vi "Test Assert Event to JSON.vi"(9 "indent level":i32, 10 "Test Event":T1={"Name"="", "Passed"=FALSE, "Call Chain"=[], "Test Error"={"status"=FALSE, "code"=0, "source"=""}, "Time Stamp"=timestamp(0 s since 1904-01-01), "Unique Assert ID"="", "Test ID"="", "Execution time (s)"=-1.0, "Verbose Explanation"=""}) -> (2 "<JSON>Assertion Event":string)   [LabVIEW 2020, in "Caraya.lvlib" / "Test Result.lvclass"]
uses:
  Test Result.lvclass
  Assert Event Data.ctl
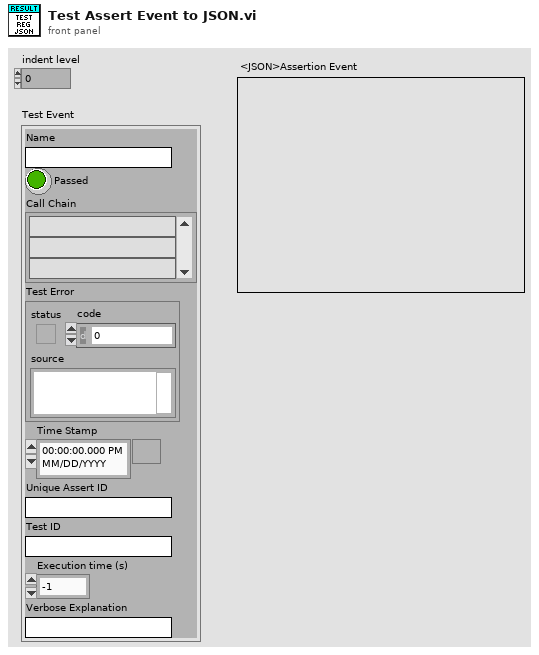
[diagram p1: front panel]
types:
  T1 = typedef "Caraya.lvlib/Test Result.lvclass/Assert Event Data.ctl" = cluster{"Name":string, "Passed":bool, "Call Chain":string[], "Test Error":errorcluster, "Time Stamp":timestamp, "Unique Assert ID":string, "Test ID":string, "Execution time (s)":dbl, "Verbose Explanation":string}
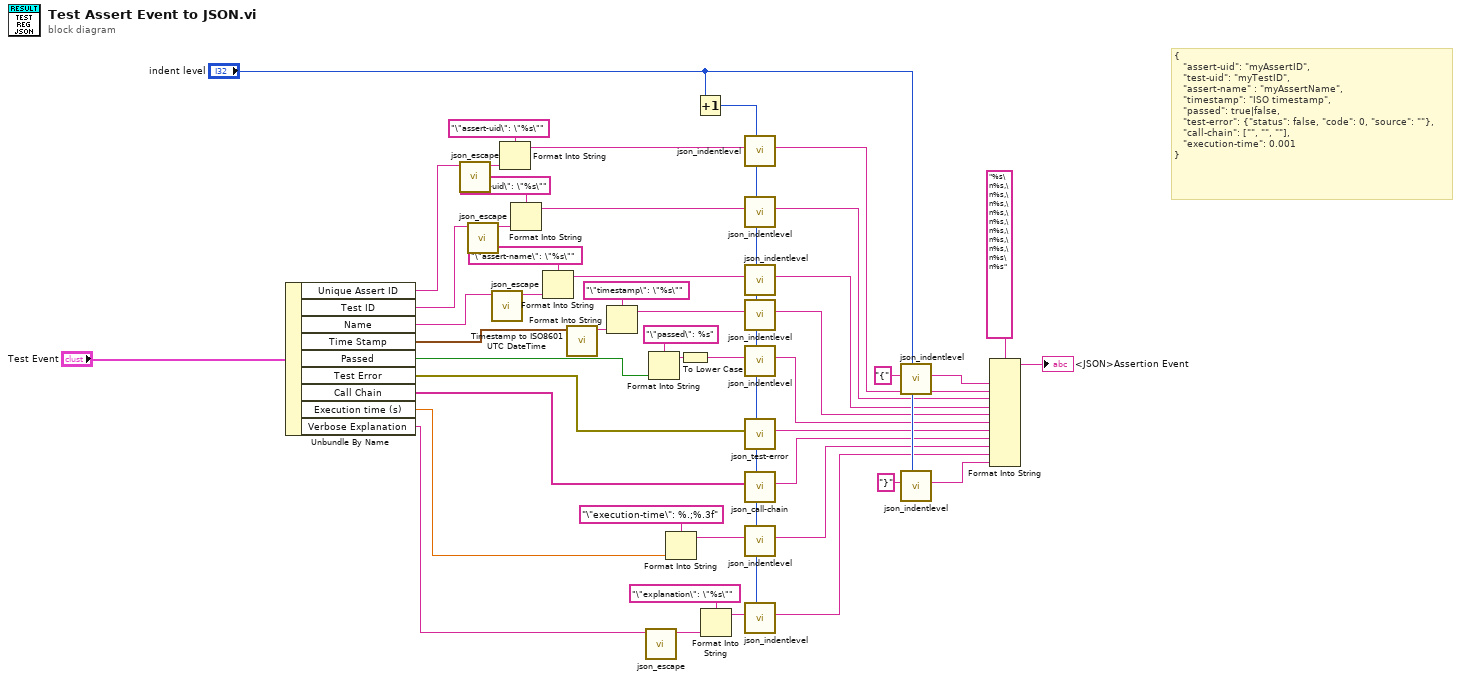
[diagram p0: block diagram]
diagram:
  # "{\n   \"assert-uid\": \"myAssertID\",\n   \"test-uid\": \"myTestID\",\n   \"assert-name\" : \"myAssertName\",\n   \"timestamp\": \"ISO timestamp\",\n   \"passed\": true|false,\n   \"test-error\": {\"status\": false, \"code\": 0, \"source\": \"\"},\n   \"call-chain\": [\"\", \"\", \"\"],\n   \"execution-time\": 0.001\n}"
  n1 = Unbundle By Name("Test Event") -> ("Unique Assert ID"=w32:string, "Test ID"=w28:string, "Name"=w24:string, "Time Stamp"=w45:timestamp, "Passed"=w18:bool, "Test Error"=w5:errorcluster, "Call Chain"=w6:string[], "Execution time (s)"=w8:dbl, "Verbose Explanation"=w12:string)
  n2 = call "json_escape.vi"("string"=w32) -> ("escaped string"=w31:string)  [unwired: 10 in]
  n3 = call "json_escape.vi"("string"=w28) -> ("escaped string"=w30:string)  [unwired: 10 in]
  n4 = call "json_escape.vi"("string"=w24) -> ("escaped string"=w25:string)  [unwired: 10 in]
  n5 = Format Into String(format string="\"assert-uid\": \"%s\"", w31) -> (resulting string=w33:string)  [unwired: 2 in, 1 out]
  n6 = Format Into String(format string="\"test-uid\": \"%s\"", w30) -> (resulting string=w27:string)  [unwired: 2 in, 1 out]
  n7 = Format Into String(format string="\"assert-name\": \"%s\"", w25) -> (resulting string=w23:string)  [unwired: 2 in, 1 out]
  n8 = call <vilib>:"Timestamp to ISO8601 UTC DateTime.vi"("Timestamp (now)"=w45) -> ("ISO8601 UTC DateTime"=w22:string)  [unwired: 10 in]
  n9 = Format Into String(format string="\"timestamp\": \"%s\"", w22) -> (resulting string=w21:string)  [unwired: 2 in, 1 out]
  n10 = call "json_escape.vi"("string"=w12) -> ("escaped string"=w15:string)  [unwired: 10 in]
  n11 = Format Into String(format string="\"passed\": %s", w18) -> (resulting string=w19:string)  [unwired: 2 in, 1 out]
  n12 = Format Into String(format string="\"execution-time\": %.;%.3f", w8) -> (resulting string=w9:string)  [unwired: 2 in, 1 out]
  n13 = To Lower Case(string=w19) -> (all lower case string=w17:string)
  n14 = Increment(x="indent level") -> (x+1=w3:i32)
  n15 = Format Into String(format string="\"explanation\": \"%s\"", w15) -> (resulting string=w13:string)  [unwired: 2 in, 1 out]
  n16 = call "json_indentlevel.vi"("indent level"=w3, "string"=w33) -> ("indented string"=w39:string)  [unwired: 9 in]
  n17 = call "json_indentlevel.vi"("indent level"=w3, "string"=w27) -> ("indented string"=w38:string)  [unwired: 9 in]
  n18 = call "json_indentlevel.vi"("indent level"=w3, "string"=w23) -> ("indented string"=w37:string)  [unwired: 9 in]
  n19 = call "json_indentlevel.vi"("indent level"=w3, "string"=w21) -> ("indented string"=w36:string)  [unwired: 9 in]
  n20 = call "json_indentlevel.vi"("indent level"=w3, "string"=w17) -> ("indented string"=w35:string)  [unwired: 9 in]
  n21 = call "json_test-error.vi"("indent level"=w3, "error"=w5) -> ("indented string"=w2:string)  [unwired: 9 in]
  n22 = call "json_call-chain.vi"("indent level"=w3, "Call Chain"=w6) -> ("indented string"=w4:string)  [unwired: 9 in]
  n23 = call "json_indentlevel.vi"("indent level"=w3, "string"=w9) -> ("indented string"=w7:string)  [unwired: 9 in]
  n24 = call "json_indentlevel.vi"("indent level"=w3, "string"=w13) -> ("indented string"=w11:string)  [unwired: 9 in]
  n25 = call "json_indentlevel.vi"("indent level"="indent level", "string"="{") -> ("indented string"=w43:string)  [unwired: 9 in]
  n26 = call "json_indentlevel.vi"("indent level"="indent level", "string"="}") -> ("indented string"=w41:string)  [unwired: 9 in]
  n27 = Format Into String(format string="%s\n%s,\n%s,\n%s,\n%s,\n%s,\n%s,\n%s,\n%s,\n%s\n%s", w43, w39, w38, w37, w36, w35, w2, w4, w7, w11, w41) -> (resulting string=→"<JSON>Assertion Event":string)  [unwired: 2 in, 1 out]
